vi "Prcess Data.vi"(8 "error in (no error)":errorcluster, 9 "Running":refnum<vi>, 10 "XY Plot":refnum<vi>, 11 "3way Lap":refnum<class "3way Lap.lvclass">) -> (0 "error out":errorcluster, 3 "3way Lap out":refnum<class "3way Lap.lvclass">)   [LabVIEW 2025, in "Flow Grind.lvlib" / "3way Lap.lvclass"]
uses:
  3way Lap.lvclass
  3way Lap.lvclass/3way Lap.ctl
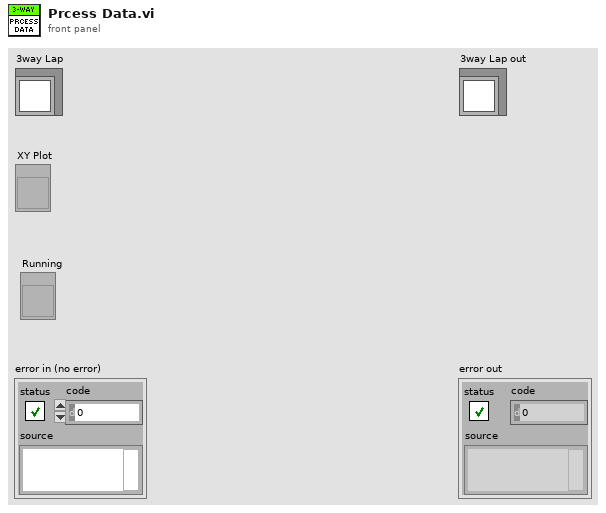
[diagram p1: front panel]
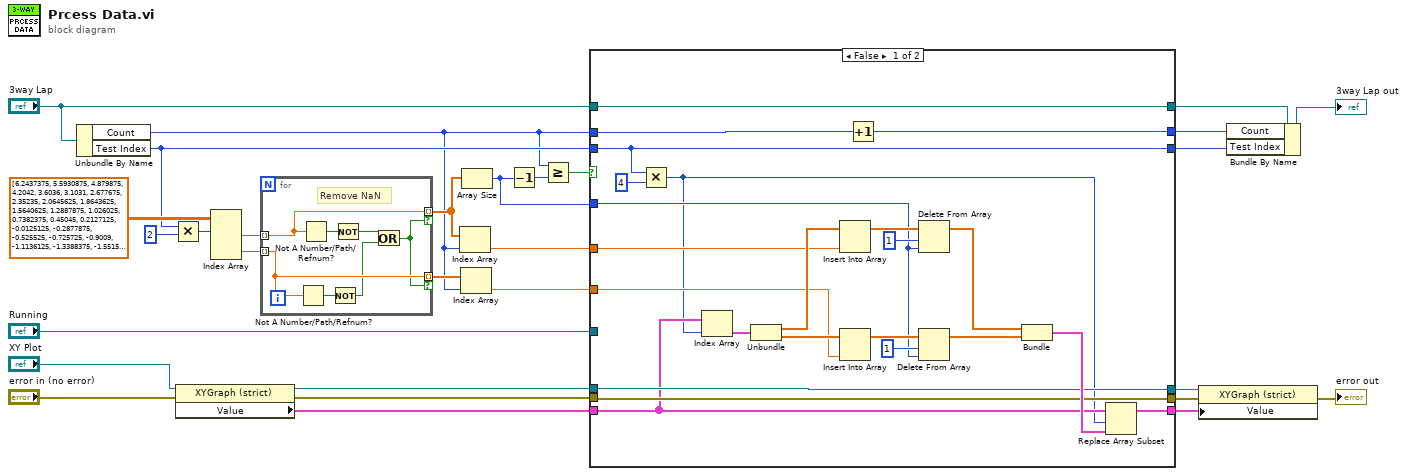
[diagram p0: block diagram]
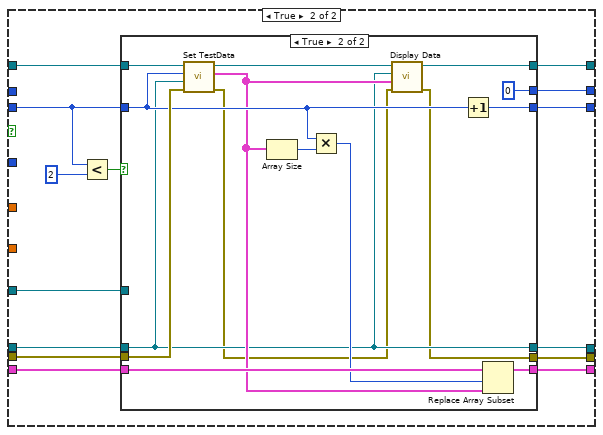
[diagram p2: hidden frame]
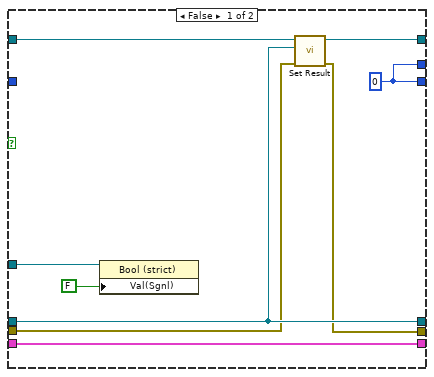
[diagram p3: hidden frame]
diagram:
  n1 = Unbundle By Name("3way Lap") -> ("Count"=w4:i32, "Test Index"=w5:u32)
  n2 = Multiply(x=w5, y=2 ("index (row)")) -> (x*y=w29:u32)
  n3 = property class="XYGraph (strict)"(reference="XY Plot", error in="error in (no error)") -> (reference out=w9:refnum<vi>, error out=w14:errorcluster, "Value"=w13:cluster{dbl[], dbl[]}[])
  n4 = Index Array(array=dbl[][] [[6.2437375, 5.5930875, 4.879875, 4.2042, 3.6036, 3.1031, 2.677675, 2.35235, 2.0645625, 1.8643625, 1.5640625, 1.2887875, 1.026025, 0.7382375, 0.45045, 0.2127125, -0.0125125, -0.2877875, -0.525525, -0.725725, -0.9009, -1.1136125, -1.3388375, -1.55155, -1.7892875, -1.95195, -2.1396375, -2.3398375, -2.627625, -2.9154125, -3.3033, -3.6661625, -3.9914875, -4.329325, -4.679675, -5.0425375, -5.4054, -5.7432375, -6.0685625, -6.2937875, -6.431425, -6.4689625, nan, nan, nan, nan, nan, nan, nan, nan, nan, nan, nan, nan, nan, nan, nan, nan, nan, nan, nan, nan, nan, nan, nan, nan, nan, nan], [4.746529, 4.0505754, 3.2230983, 2.4606815, 1.7803933, 1.237849, 0.7845591, 0.4032021, 0.0992629, -0.1124343, -0.3017973, -0.3600225, -0.3816774, -0.3988502, -0.4412808, -0.4975515, -0.498804, -0.5093461, -0.5234096, -0.5402439, -0.5895036, -0.6693163, -0.7678891, -0.9169929, -1.0808247, -1.2792367, -1.4056172, -1.6142892, -1.8344676, -2.0964115, -2.4953858, -2.6851412, -2.9267374, -3.205667, -3.5138337, -3.8592935, -4.0989134, -4.3954103, -4.6875921, -5.2416416, -5.4093912, -5.4257957, nan, nan, nan, nan, nan, nan, nan, nan, nan, nan, nan, nan, nan, nan, nan, nan, nan, nan, nan, nan, nan, nan, nan, nan, nan, nan], [6.8193125, 6.1061, 5.1926875, 4.2167125, 3.3158125, 2.6651625, 2.1146125, 1.7392375, 1.4889875, 1.276275, 1.026025, 0.7632625, 0.55055, 0.25025, nan, -0.2877875, -0.575575, -0.875875, -1.076075, -1.3388375, -1.576575, -1.85185, -2.2022, -2.55255, -2.9654625, -3.5160125, -4.1666625, -4.779775, -5.3178125, -5.85585, -6.2687625, -6.4689625, -6.4689625, -6.4689625, nan, nan, nan, nan, nan, nan, nan, nan, nan, nan, nan, nan, nan, nan, nan, nan, nan, nan, nan, nan, nan, nan, nan, nan, nan, nan, nan, nan, nan, nan, nan, nan, nan, nan], [-5.722515, -4.9150748, -3.9996873, -2.9526658, -2.1107265, -1.4969717, -1.0407705, -0.8008192, -0.6596329, -0.5810512, -0.5293486, -0.4767964, -0.4515365, -0.4295943, -0.4202443, -0.4036431, -0.3832887, -0.355239, -0.3314576, -0.119446, 0.3648198, 0.7030289, 1.0982102, 1.5460286, 1.9877319, 2.6519719, 3.4226937, 4.0790668, 4.7565556, 5.3762199, 5.8632065, 6.0722586, 6.084077, 6.0993648, nan, nan, nan, nan, nan, nan, nan, nan, nan, nan, nan, nan, nan, nan, nan, nan, nan, nan, nan, nan, nan, nan, nan, nan, nan, nan, nan, nan, nan, nan, nan, nan, nan, nan]] ("array1"), index (row) #1=w29) -> (element #1=w26:dbl[], element #2=w25:dbl[])  [unwired: 3 in]
  n5 = for {
    tunnel: w26 -> [w36] mode=indexing
    tunnel: w25 -> [w33] mode=indexing
    tunnel: [w36] -> w22 mode=indexing if=w30
    tunnel: [w33] -> w24 mode=indexing if=w30
    # "Remove NaN"
    n6 = Not A Number/Path/Refnum?(number/path/refnum=w33) -> (NaN/Path/Refnum?=w34:bool)
    n7 = Not A Number/Path/Refnum?(number/path/refnum=w36) -> (NaN/Path/Refnum?=w35:bool)
    n8 = Not(x=w34) -> (.not. x?=w32:bool)
    n9 = Not(x=w35) -> (.not. x?=w31:bool)
    n10 = Or(x=w31, y=w32) -> (x .or. y?=w30:bool)
  }
  n11 = Index Array(array=w22, index=w4) -> (element=w20:dbl)
  n12 = Index Array(array=w24, index=w4) -> (element=w19:dbl)
  n13 = Array Size(array=w22) -> (size(s)=w6:i32)
  n14 = Decrement(x=w6) -> (x-1=w23:i32)
  n15 = Greater Or Equal?(x=w4, y=w23) -> (x >= y?=w21:bool)
  n16 = case shown="False" w21 {
    tunnel: w20 -> [w43 _]
    tunnel: w19 -> [w44 _]
    tunnel: "3way Lap" -> [w59 w68]
    tunnel: [w59 w66] -> w17
    tunnel: w14 -> [w48 w64]
    tunnel: w13 -> [w45 w61]
    tunnel: [w41 w65] -> w11
    tunnel: [w48 w63] -> w10
    tunnel: w9 -> [w47 w67]
    tunnel: [w47 w62] -> w8
    tunnel: [w46 w60] -> w7
    tunnel: w6 -> [w42 _]
    tunnel: w5 -> [w39 w69]
    tunnel: w4 -> [w40 _]
    tunnel: [w39 w70] -> w3
    tunnel: "Running" -> [_ w71]
    frame False {
      n17 = Multiply(x=w39, y=4 ("index")) -> (x*y=w37:u32)
      n18 = Index Array(array=w45, index=w37) -> (element=w57:cluster{dbl[], dbl[]})
      n19 = Unbundle(w57) -> (w55:dbl[], w56:dbl[])
      n20 = Insert Into Array(array=w55, new element=w43) -> (w52:dbl[])  [unwired: 1 in]
      n21 = Insert Into Array(array=w56, new element=w44) -> (w53:dbl[])  [unwired: 1 in]
      n22 = Increment(x=w40) -> (x+1=w41:i32)
      n23 = Delete From Array(array=w52, length=1, index=w42) -> (array with subset deleted=w50:dbl[])  [unwired: 1 out]
      n24 = Delete From Array(array=w53, length=1, index=w42) -> (array with subset deleted=w49:dbl[])  [unwired: 1 out]
      n25 = Bundle(w50, w49) -> (w58:cluster{dbl[], dbl[]})  [unwired: 1 in]
      n26 = Replace Array Subset(array=w45, new element=w58, index=w37) -> (w46:cluster{dbl[], dbl[]}[])
    }
    frame True {
      n27 = Less?(x=w69, y=u32 2) -> (x < y?=w72:bool)
      n28 = case shown="True" w72 {
        tunnel: w71 -> [w82 _]
        tunnel: [w80 w97] -> w70
        tunnel: w69 -> [_ w90]
        tunnel: w68 -> [w78 w96]
        tunnel: w67 -> [w76 w85]
        tunnel: [w77 w87] -> w66
        tunnel: [w80 0] -> w65
        tunnel: w64 -> [w75 w94]
        tunnel: [w74 w83] -> w63
        tunnel: [w76 w85] -> w62
        tunnel: w61 -> [w79 w93]
        tunnel: [w79 w92] -> w60
        frame False {
          w80 = u32 0
          n29 = property class="Bool (strict)"(reference=w82, "Val(Sgnl)"=FALSE ("Value (Signaling)")) -> ()  [unwired: 1 in, 2 out]
          n30 = call "Set Result.vi"("error in (no error)"=w75, "XY Plot"=w76, "3way Lap in"=w78) -> ("error out"=w74:errorcluster, "3way Lap out"=w77:refnum<class "3way Lap.lvclass">)  [unwired: 7 in]
        }
        frame True {
          n31 = call "Set TestData.vi"("error in (no error)"=w94, "Main"=w85, "Test Index"=w90, "3way Lap In"=w96) -> ("error out"=w84:errorcluster, "Test Data"=w86:cluster{"Best Linear Fit":dbl[], "Y":dbl[]}[], "3way Lap  out"=w88:refnum<class "3way Lap.lvclass">)  [unwired: 5 in]
          n32 = Array Size(array=w86) -> (size(s)=w91:i32)
          n33 = Multiply(x=w90, y=w91) -> (x*y=w89:u32)
          n34 = call "Display Data.vi"("error in (no error)"=w84, "Test Data"=w86, "XY Plot"=w85, "3way Lap in"=w88) -> ("error out"=w83:errorcluster, "3way Lap out"=w87:refnum<class "3way Lap.lvclass">)  [unwired: 6 in]
          n35 = Increment(x=w90) -> (x+1=w97:u32)
          n36 = Replace Array Subset(array=w93, new element=w86, index=w89) -> (w92:cluster{dbl[], dbl[]}[])
        }
      }
    }
  }
  n37 = property class="XYGraph (strict)"(reference=w8, error in=w10, "Value"=w7) -> (error out=→"error out":errorcluster)  [unwired: 1 out]
  n38 = Bundle By Name(cluster=w17, "Count"=w11, "Test Index"=w3) -> (→"3way Lap out":refnum<class "3way Lap.lvclass">)
